vi "Interlock_status.vi"(8 "error in (no error)":errorcluster, 11 "VISA resource name":refnum<visa-resource-name>) -> (0 "error out":errorcluster, 3 "INTERLOCK STATUS":bool)   [LabVIEW 2021]
uses:
  GPT-9800_GSB_L8.5/GPT-9000.lvlib
panel:
  out "substring":string
  out "concatenated string":string
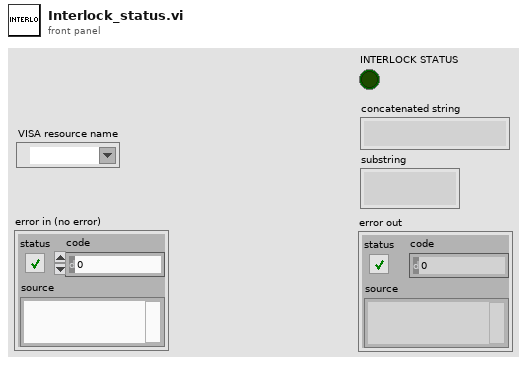
[diagram p1: front panel]
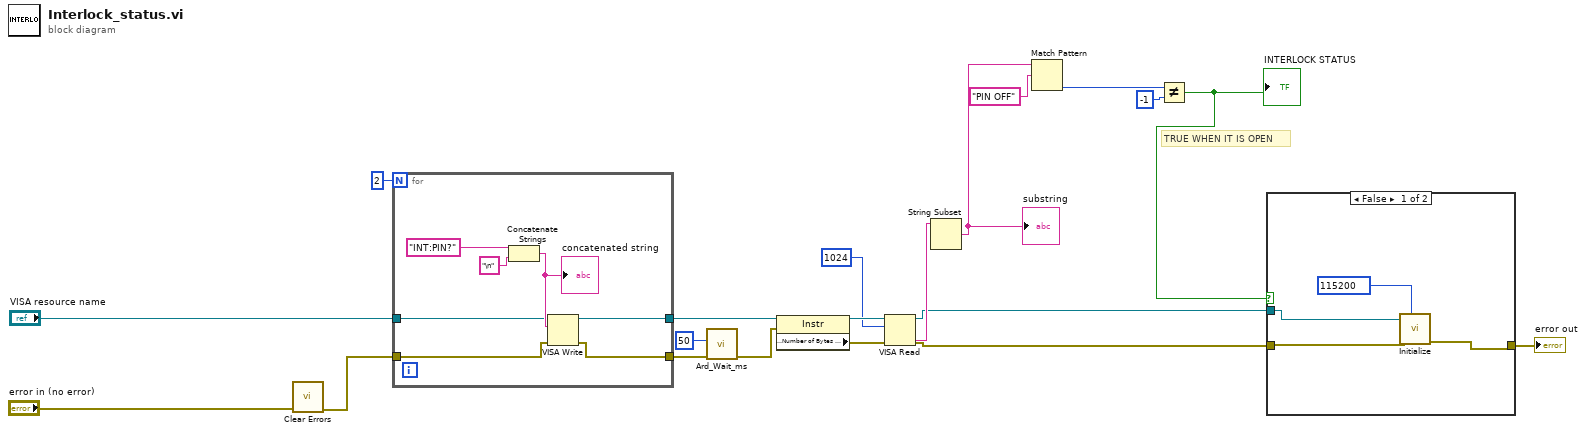
[diagram p0: block diagram]
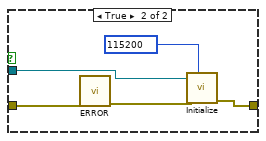
[diagram p2: hidden frame]
diagram:
  # "TRUE WHEN IT IS OPEN"
  n1 = call <vilib>:"Clear Errors.vi"("error in (no error)"="error in (no error)") -> ("error out"=w8:errorcluster)  [unwired: 5 in, 1 out]
  n2 = for {
    N: 2 -> [_]
    tunnel: "VISA resource name" -> [w22]
    tunnel: [w27] -> w18
    tunnel: w8 -> [w21]
    tunnel: [w25] -> w16
    n3 = Concatenate Strings("INT:PIN?", "\n" ("string")) -> (w26:string)
    "concatenated string" <- w26
    n4 = VISA Write(VISA resource name=w22, write buffer=w26, error in (no error)=w21) -> (VISA resource name out=w27:refnum<visa-resource-name>, error out=w25:errorcluster)  [unwired: 1 out]
  }
  n5 = call "Ard_Wait_ms.vi"("error in"=w16, "millisec"=u32 50) -> ("error in 2"=w15:errorcluster)  [unwired: 9 in]
  n6 = property class="Instr" props=["Serial Settings:Number of Bytes at Serial Port"](reference=w18, error in=w15) -> (reference out=w19:refnum<visa-resource-name>, error out=w20:errorcluster)  [unwired: 1 out]
  n7 = VISA Read(VISA resource name=w19, byte count=u32 1024, error in (no error)=w20) -> (VISA resource name out=w4:refnum<visa-resource-name>, read buffer=w14:string, error out=w6:errorcluster)  [unwired: 1 out]
  n8 = String Subset(string=w14) -> (substring=w9:string)  [unwired: 2 in]
  "substring" <- w9
  n9 = Match Pattern(string=w9, regular expression="PIN OFF") -> (offset past match=w11:i32)  [unwired: 1 in, 3 out]
  n10 = Not Equal?(x=w11, y=-1) -> (x != y?=w5:bool)
  "INTERLOCK STATUS" <- w5
  n11 = case shown="False" w5 {
    tunnel: [w28 w34] -> w7
    tunnel: w6 -> [w30 w33]
    tunnel: w4 -> [w29 w32]
    frame False {
      w31 = u32 115200 items=["9600"=9600, "19200"=19200, "38400"=38400, "57600"=57600, "115200"=115200] ("Configure RS232 Baud Rate")
      n12 = call "Initialize.vi"("Configure RS232 Baud Rate"=w31, "error in (no error)"=w30, "VISA resource name"=w29) -> ("error out"=w28:errorcluster)  [unwired: 5 in, 3 out]
    }
    frame True {
      w35 = u32 115200 items=["9600"=9600, "19200"=19200, "38400"=38400, "57600"=57600, "115200"=115200] ("Configure RS232 Baud Rate")
      n13 = call "ERROR.vi"(8:w33) -> ("error"=w36:errorcluster)  [unwired: 10 in]
      n14 = call "Initialize.vi"("Configure RS232 Baud Rate"=w35, "error in (no error)"=w36, "VISA resource name"=w32) -> ("error out"=w34:errorcluster)  [unwired: 5 in, 3 out]
    }
  }
  "error out" <- w7
